vi "GetCacheFolder.vi"(8 "error in (no error)":errorcluster) -> (0 "error out":errorcluster, 3 "cache folder":path)   [LabVIEW 2023, in "GettingStartedWindow.lvlib" / "Feed_link.lvclass"]
uses:
  <resource>/modes/FRC/GSW/Classes/Feed_link/Feed_link.lvclass
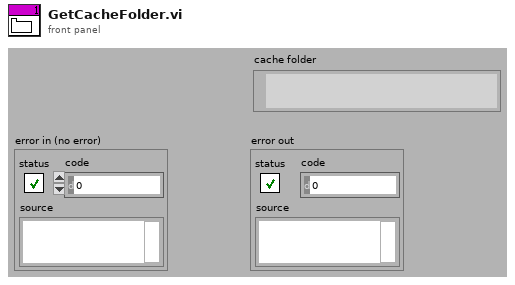
[diagram p1: front panel]
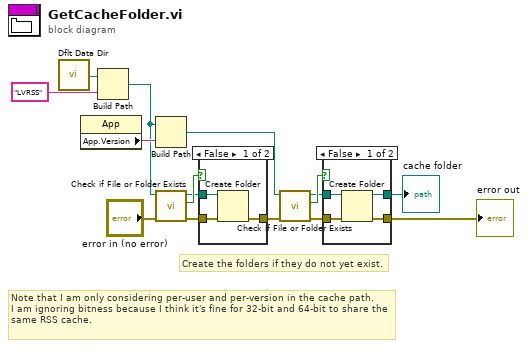
[diagram p0: block diagram]
diagram:
  # "Create the folders if they do not yet exist."
  # "Note that I am only considering per-user and per-version in the cache path. \nI am ignoring bitness because I think it's fine for 32-bit and 64-bit to share the\nsame RSS cache."
  n1 = call <vilib>:"Dflt Data Dir.vi"() -> ("App:Default Data Directory"=w15:path)
  n2 = property class="App"() -> ("App.Version"=w13:string)  [unwired: 2 in, 2 out]
  n3 = Build Path(base path=w15, name or relative path="LVRSS") -> (appended path=w12:path)
  n4 = Build Path(base path=w12, name or relative path=w13) -> (appended path=w7:path)
  n5 = call <vilib>:"Check if File or Folder Exists.vi"("error in (no error)"="error in (no error)", "path"=w12) -> ("error out"=w9:errorcluster, "file or folder exists?"=w11:bool, "dup path"=w10:path)  [unwired: 7 out]
  n6 = case shown="False" w11 {
    tunnel: w10 -> [w18 _]
    tunnel: w9 -> [w17 w19]
    tunnel: [w16 w19] -> w3
    frame False {
      n7 = Create Folder(path (use dialog)=w18, error in=w17) -> (error out=w16:errorcluster)  [unwired: 3 out]
    }
    frame True {
    }
  }
  n8 = call <vilib>:"Check if File or Folder Exists.vi"("error in (no error)"=w3, "path"=w7) -> ("error out"=w4:errorcluster, "file or folder exists?"=w6:bool, "dup path"=w5:path)  [unwired: 7 out]
  n9 = case shown="False" w6 {
    tunnel: w5 -> [w23 w24]
    tunnel: w4 -> [w22 w25]
    tunnel: [w21 w25] -> w1
    tunnel: [w20 w24] -> w2
    frame False {
      n10 = Create Folder(path (use dialog)=w23, error in=w22) -> (created path=w20:path, error out=w21:errorcluster)  [unwired: 2 out]
    }
    frame True {
    }
  }
  "cache folder" <- w2
  "error out" <- w1
